vi "Acquire.vi"(8 "error in (no error)":errorcluster, 11 "Buffer in":refnum<class "Buffer.lvclass">) -> (0 "error out":errorcluster, 3 "Mapped Buffer":refnum<data-value>)   [LabVIEW 2020, in "Buffer Byte-Stream Access.lvclass"]
uses:
  Buffer Byte-Stream Access.lvclass
  Buffer/Buffer.lvclass
  Buffer/Buffer.lvclass/Buffer.ctl
  Image Info.ctl
  Buffer Byte-Stream Access.lvclass/Buffer Byte-Stream Access.ctl
  bin/gindustrialcam_32-1.dll
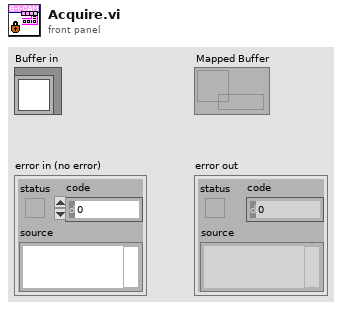
[diagram p1: front panel]
types:
  T1 = typedef "Buffer Byte-Stream Access.lvclass/Image Info.ctl" = cluster{"X Resolution":i32, "Y Resolution":i32, "Bytes to Copy":u64}
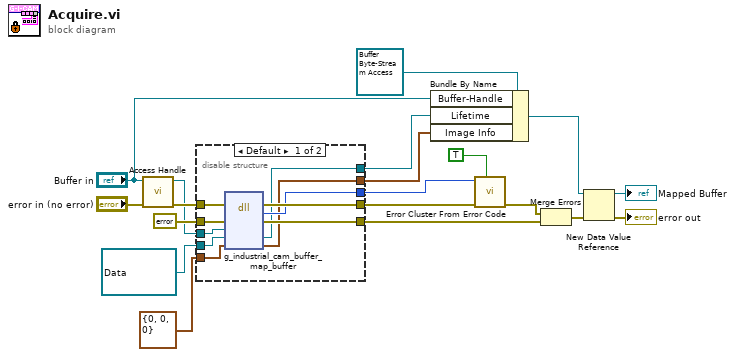
[diagram p0: block diagram]
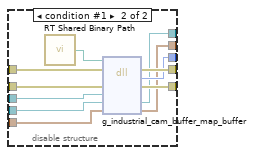
[diagram p2: hidden frame]
diagram:
  n1 = call "Access Handle.vi"("error in (no error)"="error in (no error)", "Buffer"="Buffer in") -> ("error out"=w7:errorcluster, "Handle"=w6:refnum<data-value>)  [unwired: 8 in]
  n2 = disable-structure shown="Default" {
    disable-tunnel: [w29 w40] -> w13
    disable-tunnel: [w28 w39] -> w12
    disable-tunnel: [w27 w38] -> w10
    disable-tunnel: errorcluster {"status"=FALSE, "code"=0, "source"=""} ("error constant") -> [w26 w37]
    disable-tunnel: w7 -> [w25 w36]
    disable-tunnel: w6 -> [w24 w35]
    disable-tunnel: refnum<data-value> refnum ("Lifetime") -> [w23 w34]
    disable-tunnel: [w22 w33] -> w4
    disable-tunnel: T1 {"X Resolution"=0, "Y Resolution"=0, "Bytes to Copy"=0} ("Image Info") -> [w21 w32]
    disable-tunnel: [w20 w31] -> w2
    frame condition #0 (active) {
      n3 = dll-call lib="C:/serenial/lib/g-industrial-camera/LabVIEW/g_industrial_cam/bin/gindustrialcam_*-1.*" fn="g_industrial_cam_buffer_map_buffer"(error in=w25, "err"=w26, "buffer_handle"=w24, "lifetime_edvr"=w23, "info_ptr"=w21) -> (error out=w29:errorcluster, "Mg_Error"=w28:i32, "err"=w27:errorcluster, "lifetime_edvr"=w22:refnum<data-value>, "info_ptr"=w20:T1)  [unwired: 3 in, 1 out]
    }
    frame condition #1 {
      n4 = call "RT Shared Binary Path.vi"() -> ("Path"=w30:path)
      n5 = dll-call lib="C:/serenial/lib/g-industrial-camera/LabVIEW/g_industrial_cam/bin/gindustrialcam_*-1.*" fn="g_industrial_cam_buffer_map_buffer"(path in=w30, error in=w36, "err"=w37, "buffer_handle"=w35, "lifetime_edvr"=w34, "info_ptr"=w32) -> (error out=w40:errorcluster, "Mg_Error"=w39:i32, "err"=w38:errorcluster, "lifetime_edvr"=w33:refnum<data-value>, "info_ptr"=w31:T1)  [unwired: 2 in, 1 out]
    }
  }
  n6 = Bundle By Name(cluster=refnum<class "Buffer Byte-Stream Access.lvclass"> refnum ("Buffer-Mapped.lvclass"), "Buffer-Handle"="Buffer in", "Lifetime"=w4, "Image Info"=w2) -> (w17:refnum<class "Buffer Byte-Stream Access.lvclass">)
  n7 = call <vilib>:"Error Cluster From Error Code.vi"("show call chain? (False)"=TRUE, "error in (no error)"=w13, "error code (0)"=w12) -> ("error out"=w11:errorcluster)  [unwired: 6 in]
  n8 = Merge Errors(w11, w10) -> (w1:errorcluster)
  n9 = New Data Value Reference(data value=w17, error in=w1) -> (data value reference=→"Mapped Buffer":refnum<data-value>, error out=→"error out":errorcluster)
